vi "Measure.vi"(8 "error in (no error)":errorcluster, 9 "measurement configuration":variant, 10 "measure call context in":refnum<class "Measure Call Context.lvclass">, 11 "measurement plugin in":refnum<class "Automotive Vision.lvclass">) -> (0 "error out":errorcluster, 1 "measurement results":variant, 2 "measure call context out":refnum<class "Measure Call Context.lvclass">, 3 "measurement plugin out":refnum<class "Automotive Vision.lvclass">)   [LabVIEW 2025, in "Automotive Vision.lvclass"]
uses:
  Automotive Vision.lvclass
  Automotive Vision.lvclass/Automotive Vision.ctl
  Measurement Configuration.ctl
  Automotive-Vision OOB Data Transfer/Automotive-Vision OOB Data Transfer.lvlib
  Automotive-Vision-OOBService_server/Automotive-Vision-OOBService_server.lvlib
  <vilib>/Plug-In SDKs/Measurements/Measure Call Context/Measure Call Context.lvclass
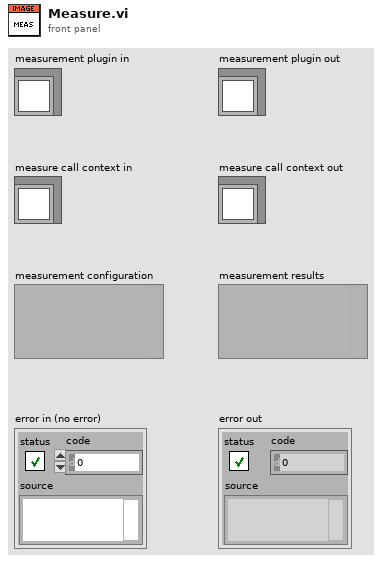
[diagram p1: front panel]
types:
  T1 = typedef "Automotive Vision.lvclass/Measurement Configuration.ctl" = cluster{"config":string, "bitfile":string}
  T2 = typedef "Automotive Vision.lvclass/Measurement Results.ctl" = cluster{"ACQ. IN PROGRESS":bool, "IMAGE PIXEL DATA":u32[], "ACQ. DURATION (s)":dbl, "SOURCE RATE (fps)":dbl, "BYTES ACQUIRED":u64, "FRAME COUNT":u64, "POC VOLTAGE (V)":dbl, "POC CURRENT (A)":dbl, "ERROR":bool, "STATE MESSAGE":string, "IMAGE DATA":string, "OOB gRPC Port":i32, "HEIGHT":u64, "WIDTH":u64}
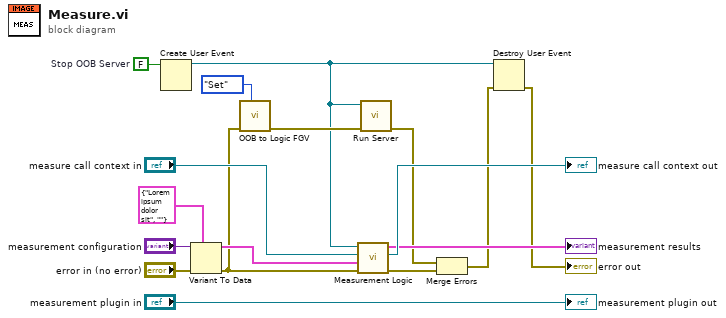
[diagram p0: block diagram]
diagram:
  w9 = FALSE  # Stop OOB Server
  n1 = Create User Event(user event datatype=w9) -> (user event=w1:refnum<user-event>)  [unwired: 1 in, 1 out]
  n2 = Variant To Data(error in="error in (no error)", type=T1 {"config"="Lorem ipsum dolor sit", "bitfile"=""} ("measurement configuration"), Variant="measurement configuration") -> (data=w11:T1, error out=w8:errorcluster)
  n3 = call "OOB to Logic FGV.vi"("Op (Get)"=enum16{"Get", "Set"}."Set", "error in (no error)"=w8) -> ("error out"=w6:errorcluster)  [unwired: 8 in, 1 out]
  n4 = call "Measurement Logic.vi"("error in"=w8, "measurement configuration"=w11, "measure call context in"="measure call context in", "user event out"=w1) -> ("Error Out"=w5:errorcluster, "measure call context out"=→"measure call context out":refnum<class "Measure Call Context.lvclass">, "measurement results"=→"measurement results":T2)  [unwired: 5 in]
  n5 = call "Run Server.vi"("error in (no error)"=w6, "Stop OOB Server UE"=w1) -> ("error out"=w4:errorcluster)  [unwired: 9 in]
  n6 = Merge Errors(w4, w5) -> (w3:errorcluster)
  n7 = Destroy User Event(user event=w1, error in=w3) -> (error out=→"error out":errorcluster)
  "measurement plugin out" <- "measurement plugin in"
